vi "ReadState.vi"(8 "error in (no error)":errorcluster, 11 "Viewmodel in":refnum<class "Viewmodel.lvclass">) -> (0 "error out":errorcluster, 2 "State":T1, 3 "Viewmodel out":refnum<class "Viewmodel.lvclass">)   [LabVIEW 2024, in "Viewmodel.lvclass"]
uses:
  Viewmodel.lvclass
  State.ctl
  Viewmodel.lvclass/Viewmodel.ctl
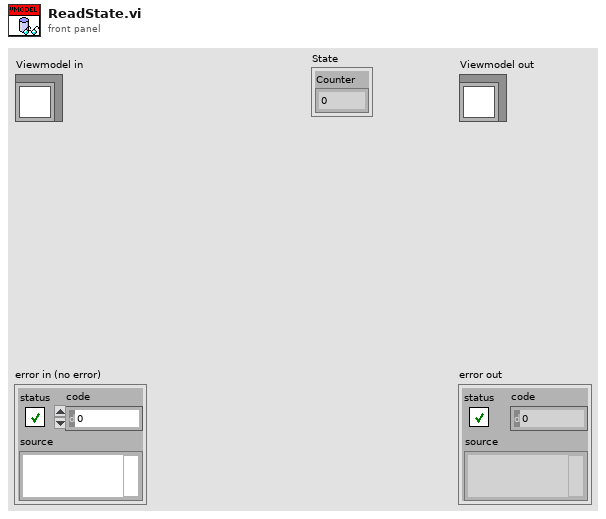
[diagram p1: front panel]
types:
  T1 = typedef "Viewmodel.lvclass/State.ctl" = cluster{"Counter":i32}
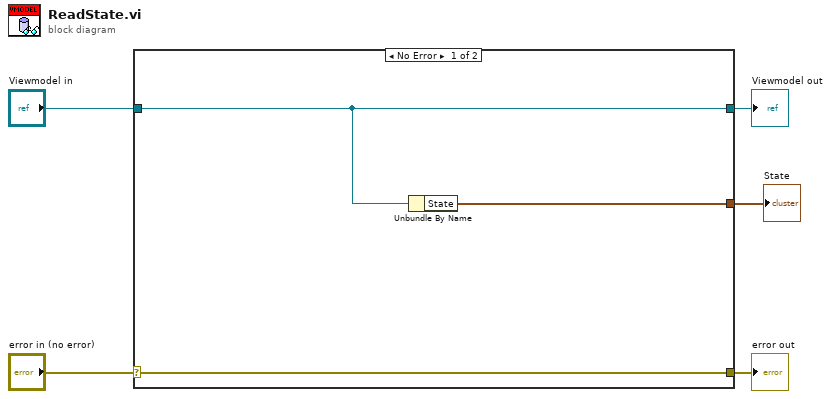
[diagram p0: block diagram]
diagram:
  n1 = case shown="No Error" "error in (no error)" {
    selector: "error in (no error)" -> [w8 w10]
    tunnel: [w8 w10] -> w4
    tunnel: [w7 w9] -> w2
    tunnel: "Viewmodel in" -> [w7 w9]
    tunnel: [w6 _] -> w1
    frame No Error {
      n2 = Unbundle By Name(w7) -> ("State"=w6:T1)
    }
    frame Error {
    }
  }
  "error out" <- w4
  "Viewmodel out" <- w2
  "State" <- w1
